vi "macro_HolDrvController_ExecuteSP.vi"() -> ()   [LabVIEW 2019, in "Trajectory_Library.lvlib"]
uses:
  Trajectory_Library.lvlib
  TypeDef/POSE2D.ctl
  TypeDef/TRANSLATION2D.ctl
  TypeDef/ROTATION2D.ctl
  TypeDef/CHASSIS_SPEEDS.ctl
  Pose2d_New.vi
  Conv_Deg_Radians.vi
  ProfiledPIDController_NewPeriod.vi
  ProfiledPIDController_SetIntegratorRange.vi
  ProfiledPIDController_DisableContInput.vi
  ProfiledPIDController_EnableContInput.vi
  TrapProfConstraint_New.vi
  HolDrvCtrl_New.vi
  HolDrvCtrl_PackPID.vi
  HolDrvCtrl_SetTolerance.vi
  HolDrvCtrl_SetEnabled.vi
  HolDrvCtrl_AtReference.vi
  HolDrvCtrl_Calculate.vi
  Rotation2d_CreateAngle.vi
  Translation2d_Create.vi
  TrapProfState_New.vi
  PIDController_NewPeriod.vi
  <vilib>/Rock Robotics/SystemInterfaces/NetworkCommunication/NetComm_UsageReport_report.vi
  PIDController_SetIntegratorRange.vi
  PIDController_DisableContinousInput.vi
  PIDController_EnableContinousInput.vi
  PIDController_Reset.vi
  Pose2d_getXYAngle.vi
  Rotation2d_GetRadians.vi
  Rotation2d_GetAngleCosSin.vi
  Pose2d_RelativeTo.vi
  Pose2d_getRotation.vi
  Rotation2d_Minus.vi
  ProfiledPIDController_Calculate_Meas_Goal.vi
  PIDController_Calculate_SP_PV.vi
  ProfiledPIDController_Reset_PosOnly.vi
  ChassisSpeeds_FromFieldRelativeSpeeds.vi
  Transform2d_Create_PosePose.vi
  Pose2d_New_TRRO.vi
  Rotation2d_UnaryMinus.vi
  Rotation2d_RotateBy.vi
  ProfiledPIDController_SetGoal_PosOnly.vi
  ProfiledPIDController_Calculate_Meas.vi
  PIDController_SetSetpoint.vi
  PIDController_Calculate_PV.vi
  ProfiledPIDController_Reset.vi
  Rotation2d_GetCos.vi
  Rotation2d_GetSin.vi
  ChassisSpeeds_New.vi
  Translation2d_RotateBy.vi
  Translation2d_Minus.vi
  Rotation2d_CreateXY.vi
  ProfiledPIDController_SetGoal.vi
  TrapProfile_New.vi
  ProfiledPIDController_GetPeriod.vi
  TrapProfile_Calculate.vi
  ControllerUtil_GetModulusError.vi
  Util_CalcDist.vi
  TrapProfile_ShouldFlipAcceleration.vi
  TrapProfile_Direct.vi
  PIDController_GetPeriod.vi
  Globals/Util_LibraryGlobals.vi
panel:
  out "calcChassisSpeed":T1 {"vOmega" format="%10.3f"; "vY" format="%10.3f"; "vX" format="%10.3f"}
  in  "X":dbl=0.02
  in  "Y":dbl=0.02
  in  "Heading_Deg":dbl=0.02
  in  "LinearVel":dbl=0.02
  in  "angleRef":T2={"VALUE"=0.0, "COS"=1.0, "SIN"=0.0} {"SIN" format="%13.4f"; "COS" format="%13.4f"; "VALUE" format="%13.4f"}
  in  "currentPose":T3={"TRANSLATION"={"X"=0.0, "Y"=0.0}, "ROTATION"={"VALUE"=0.0, "COS"=1.0, "SIN"=0.0}} {"ROTATION"."SIN" format="%13.4f"; "ROTATION"."COS" format="%13.4f"; "ROTATION"."VALUE" format="%13.4f"; "TRANSLATION"."Y" format="%14.3f"; "TRANSLATION"."X" format="%14.3f"}
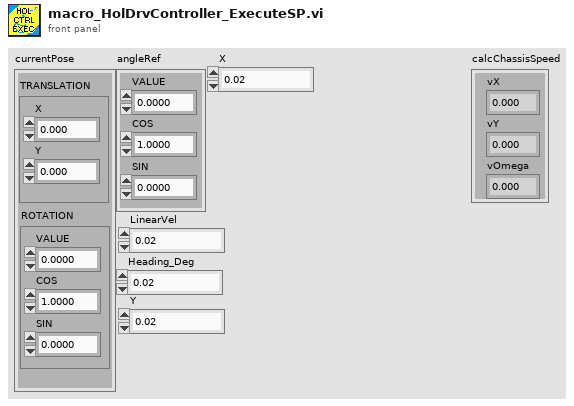
[diagram p1: front panel]
types:
  T1 = typedef "Trajectory_Library.lvlib/CHASSIS_SPEEDS.ctl" = cluster{"vX":dbl, "vY":dbl, "vOmega":dbl}
  T2 = typedef "Trajectory_Library.lvlib/ROTATION2D.ctl" = cluster{"VALUE":dbl, "COS":dbl, "SIN":dbl}
  T3 = typedef "Trajectory_Library.lvlib/POSE2D.ctl" = cluster{"TRANSLATION":T4, "ROTATION":T2}
  T4 = typedef "Trajectory_Library.lvlib/TRANSLATION2D.ctl" = cluster{"X":dbl, "Y":dbl}
  T5 = typedef "Trajectory_Library.lvlib/PID_TUNING.ctl" = cluster{"Kp":dbl, "Ki":dbl, "Kd":dbl, "MaximumIntegral":dbl, "MinimumIntegral":dbl, "IntegralZone":dbl}
  T6 = typedef "Trajectory_Library.lvlib/PROFILED_PID_CONTROLLER.ctl" = cluster{"Controller":T7, "Goal":T8, "Setpoint":T8, "Constraint":T9}
  T7 = typedef "Trajectory_Library.lvlib/PID_CONTROLLER.ctl" = cluster{"Kp":dbl, "Ki":dbl, "Kd":dbl, "Period":dbl, "Max_Integral":dbl, "Min_Integral":dbl, "Max_Input":dbl, "Min_Input":dbl, "Continuous":bool, "PositionError":dbl, "VelocityError":dbl, "PrevError":dbl, "Total_Integral":dbl, "PositionTolerance":dbl, "VelocityTolerance":dbl, "SetPoint":dbl, "Kf":dbl, "Prev_Deriv":dbl, "Prev_Deriv 2":dbl, "DerivativeFilter":bool, "Min_Output":dbl, "Max_Output":dbl, "Prev_F_P":dbl, "Prev_F_P_2":dbl, "AntiWindupActive":bool, "Measurement":dbl, "IntegralZone":dbl}
  T8 = typedef "Trajectory_Library.lvlib/TRAPEZOID_PROFILE_STATE.ctl" = cluster{"Position":dbl, "Velocity":dbl}
  T9 = typedef "Trajectory_Library.lvlib/TRAPEZOID_PROFILE_CONSTRAINT.ctl" = cluster{"MaxVelocity":dbl, "MaxAcceleration":dbl}
  T10 = typedef "Trajectory_Library.lvlib/HOLONOMIC_PACK_TUNING.ctl" = cluster{"X PID Tuning":T5, "Y PID Tuning":T5, "thetaProfiledPID_CTRL":T6}
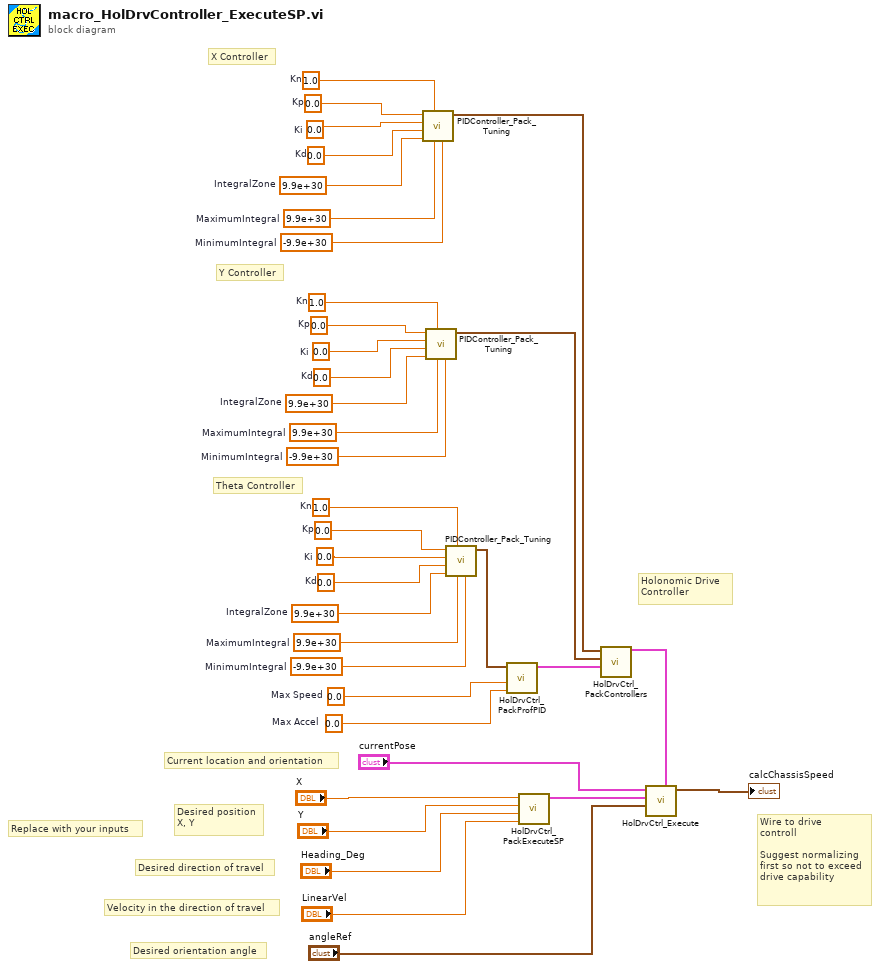
[diagram p0: block diagram]
diagram:
  w1 = 9.9e+30  # IntegralZone
  w2 = 9.9e+30  # IntegralZone
  w3 = 9.9e+30  # IntegralZone
  w31 = 1.0  # Kn
  w28 = 0.0  # Kp
  w19 = 0.0  # Ki
  w18 = 0.0  # Kd
  w17 = 9.9e+30  # MaximumIntegral
  w16 = -9.9e+30  # MinimumIntegral
  w33 = 1.0  # Kn
  w30 = 0.0  # Kp
  w27 = 0.0  # Ki
  w26 = 0.0  # Kd
  w25 = 9.9e+30  # MaximumIntegral
  w24 = -9.9e+30  # MinimumIntegral
  w32 = 1.0  # Kn
  w29 = 0.0  # Kp
  w23 = 0.0  # Ki
  w22 = 0.0  # Kd
  w21 = 9.9e+30  # MaximumIntegral
  w20 = -9.9e+30  # MinimumIntegral
  w34 = 0.0  # Max Accel
  w35 = 0.0  # Max Speed
  # "Current location and orientation"
  # "Holonomic Drive\nController"
  # "Desired orientation angle"
  # "Velocity in the direction of travel"
  # "Desired direction of travel"
  # "Desired position\nX, Y"
  # "Replace with your inputs"
  # "Wire to drive\ncontroll\n\nSuggest normalizing\nfirst so not to exceed\ndrive capability"
  # "Theta Controller"
  # "Y Controller"
  # "X Controller"
  n1 = call "PIDController_Pack_Tuning.vi"("MinimumIntegral"=w24, "MaximumIntegral"=w25, "Kn"=w33, "IntegralZone"=w3, "Kd"=w26, "Ki"=w27, "Kp"=w30) -> ("PID Tuning"=w14:T5)  [unwired: 4 in]
  n2 = call "PIDController_Pack_Tuning.vi"("MinimumIntegral"=w20, "MaximumIntegral"=w21, "Kn"=w32, "IntegralZone"=w2, "Kd"=w22, "Ki"=w23, "Kp"=w29) -> ("PID Tuning"=w12:T5)  [unwired: 4 in]
  n3 = call "PIDController_Pack_Tuning.vi"("MinimumIntegral"=w16, "MaximumIntegral"=w17, "Kn"=w31, "IntegralZone"=w1, "Kd"=w18, "Ki"=w19, "Kp"=w28) -> ("PID Tuning"=w36:T5)  [unwired: 4 in]
  n4 = call "HolDrvCtrl_PackProfPID.vi"("Max Accel"=w34, "Max Speed"=w35, "Theta PID Tuning"=w36) -> ("Theta PID CONTROLLER"=w13:T6)  [unwired: 8 in]
  n5 = call "HolDrvCtrl_PackExecuteSP.vi"("LinearVel"="LinearVel", "Heading_Deg"="Heading_Deg", "Y"="Y", "X"="X") -> ("HolExecuteSP"=w15:cluster{"DesiredPose":T3, "LinearVel":dbl})  [unwired: 7 in]
  n6 = call "HolDrvCtrl_PackControllers.vi"("thetaProfiledPID_CTRL"=w13, "Y PID Tuning"=w12, "X PID Tuning"=w14) -> ("HOLONOMIC_CTRL_PACK_TUNING"=w11:T10)  [unwired: 8 in]
  n7 = call "HolDrvCtrl_Execute.vi"("HOLONOMIC_CTRL_PACK_TUNING"=w11, "angleRef"="angleRef", "HolExecuteSP"=w15, "currentPose"="currentPose") -> ("calcChassisSpeed"=→"calcChassisSpeed":T1)  [unwired: 5 in, 2 out]
